vi "Add.vi"(8 "error in":errorcluster, 10 "Delta":dbl, 11 "Actor in":refnum<class "CounterActor.lvclass">) -> (0 "error out":errorcluster, 3 "Actor out":refnum<class "CounterActor.lvclass">)   [LabVIEW 2026, in "CounterActor.lvclass"]
doc: "Message Counter actor method: Add. Counter and Processed are private actor state."
uses:
  CounterActor.lvclass
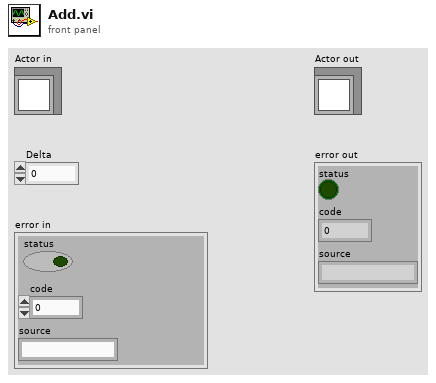
[diagram p1: front panel]
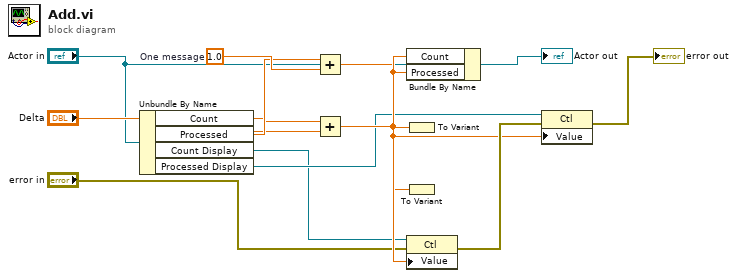
[diagram p0: block diagram]
diagram:
  w8 = 1.0  # One message
  n1 = Unbundle By Name("Actor in") -> ("Count"=w4:dbl, "Processed"=w5:dbl, "Count Display"=w6:refnum<vi>, "Processed Display"=w7:refnum<vi>)
  n2 = Add(x=w5, y=w8) -> (x+y=w9:dbl)
  n3 = Add(x=w4, y="Delta") -> (x+y=w10:dbl)
  n4 = Bundle By Name(cluster="Actor in", "Count"=w10, "Processed"=w9) -> (→"Actor out":refnum<class "CounterActor.lvclass">)
  n5 = To Variant(anything=w10) -> ()  [unwired: 1 out]
  n6 = To Variant(anything=w9) -> ()  [unwired: 1 out]
  n7 = property class="Ctl"(reference=w6, error in="error in", "Value"=w10) -> (error out=w12:errorcluster)  [unwired: 1 out]
  n8 = property class="Ctl"(reference=w7, error in=w12, "Value"=w9) -> (error out=→"error out":errorcluster)  [unwired: 1 out]
